vi "CarWashTest.vi"(0 "VI Reference In":refnum<vi>, 2 "Label":string, 5 "Wash Option":string, 7 "Car Position":i32=1, 9 "Elapsed Time":dbl=5.0, 11 "error in":errorcluster) -> (4 "VI Reference Out":refnum<vi>, 15 "error out":errorcluster)   [LabVIEW 2016, in "CarWashTest.lvlib"]
doc: "Wash test"
uses:
  CarWashTest.lvlib
  APIs/Stimulus/VI/OpenVIFrontPanel.vi
  APIs/Stimulus/ControlValue/ValueSignalByPathString.vi
  APIs/Stimulus/ControlValue/ValueSignalLatchBooleanString.vi
  APIs/Assert/AssertControlProperty/AssertControlDisable/AssertDisabledAndGrayedOut.vi
  APIs/Assert/AssertControlValue/True.vi
  APIs/Stimulus/ControlValue/SetValueAuto.vi
  APIs/Assert/AssertControlValue/Equal.vi
  APIs/Assert/AssertControlValue/AlmostEqual.vi
  <vilib>/addons/_JKI Toolkits/Caraya/classes/Assert/Assert Almost Equal_Float.vi
  Drona.lvlib
  <vilib>/addons/_JKI Toolkits/Caraya/classes/Test/Test.lvclass
  APIs/Assert/AssertControlValue/AssertControlValue.lvlib
  <vilib>/addons/_JKI Toolkits/Caraya/classes/Assert/Assert.lvclass
  APIs/Assert/AssertControlProperty/AssertControlDisable/AssertControlDisable.lvlib
  APIs/Stimulus/ControlValue/ControlValue.lvlib
  APIs/Stimulus/VI/VI.lvlib
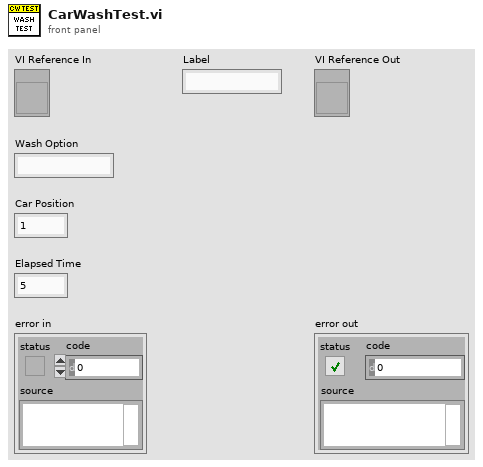
[diagram p1: front panel]
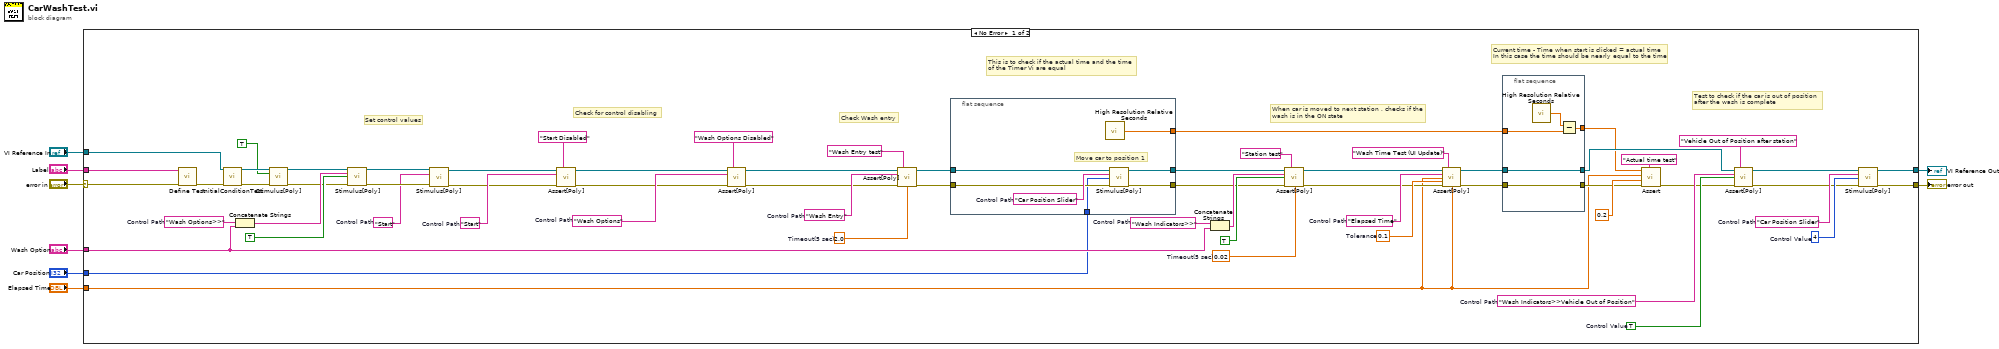
[diagram p0: block diagram]
diagram:
  n1 = case shown="No Error" "error in" {
    selector: "error in" -> [w50 w84]
    tunnel: "Wash Option" -> [w42 _]
    tunnel: "Car Position" -> [w41 _]
    tunnel: "Label" -> [w40 _]
    tunnel: "VI Reference In" -> [w36 _]
    tunnel: "Elapsed Time" -> [w26 _]
    tunnel: [w10 _] -> w2
    tunnel: [w9 w84] -> w1
    frame No Error {
      w19 = "Start"  # Control Path
      w20 = "Wash Options"  # Control Path
      w44 = "Wash Indicators>>"  # Control Path
      w45 = "Start"  # Control Path
      w49 = "Wash Options>>"  # Control Path
      w55 = 4  # Control Value
      w56 = "Car Position Slider"  # Control Path
      w59 = TRUE  # Control Value
      w66 = 0.02  # Timeout(5 sec)
      w63 = 0.1  # Tolerance
      w64 = "Elapsed Time"  # Control Path
      w60 = "Wash Indicators>>Vehicle Out of Position"  # Control Path
      w70 = 2.0  # Timeout(5 sec)
      w71 = "Wash Entry"  # Control Path
      # "Current time - Time when start is clicked = actual time\nIn this case the time should be nearly equal to the time"
      # "This is to check if the actual time and the time \nof the Timer Vi are equal"
      # "Check Wash entry"
      # "Check for control disabling"
      # "Set control values"
      # "Test to check if the car is out of position \nafter the wash is complete"
      # "When car is moved to next station , checks if the\nwash is in the ON state"
      n2 = call <vilib>:"Define Test.vi"("error in (no error)"=w50, "Label (VI Title)"=w40) -> ("error out"=w37:errorcluster)  [unwired: 8 in, 1 out]
      n3 = call "InitialConditionTest.vi"("VI Reference In"=w36, "error in"=w37) -> ("VI Reference Out"=w25:refnum<vi>, "error out"=w23:errorcluster)  [unwired: 12 in]
      n4 = Concatenate Strings(w49, w42) -> (w51:string)
      n5 = call-poly "Stimulus[Poly].vi"("VI Reference In"=w25, "Activate (F)"=TRUE ("Wait Until Done (F)"), "error in"=w23) -> ("VI Reference Out"=w24:refnum<vi>, "error out"=w22:errorcluster)  [unwired: 11 in]
      n6 = call-poly "Stimulus[Poly].vi"("VI Reference In"=w24, "Control Path"=w51, "Value (Signaling)"=TRUE, "error in"=w22) -> ("VI Reference Out"=w47:refnum<vi>, "error out"=w48:errorcluster)  [unwired: 10 in]
      n7 = call-poly "Stimulus[Poly].vi"("VI Reference In"=w47, "Control Path"=w45, "error in"=w48) -> ("VI Reference Out"=w15:refnum<vi>, "error out"=w12:errorcluster)  [unwired: 11 in]
      n8 = call-poly "Assert[Poly].vi"("VI Reference In"=w15, "Test Label"="Start Disabled", "Control Path"=w19, "Error In"=w12) -> ("VI Reference Out"=w17:refnum<vi>, "Error Out"=w18:errorcluster)  [unwired: 9 in, 1 out]
      n9 = call-poly "Assert[Poly].vi"("VI Reference In"=w17, "Test Label"="Wash Options Disabled", "Control Path"=w20, "Error In"=w18) -> ("VI Reference Out"=w14:refnum<vi>, "Error Out"=w13:errorcluster)  [unwired: 9 in, 1 out]
      n10 = call-poly "Assert[Poly].vi"("VI Reference In"=w14, "Test Label"="Wash Entry test" ("Label"), "Control Path"=w71, "Error In"=w13, "Timeout(5 sec)"=w70) -> ("VI Reference Out"=w68:refnum<vi>, "Error Out"=w69:errorcluster)  [unwired: 8 in, 1 out]
      n11 = flat-sequence {
        tunnel: w69 -> [w82]
        tunnel: w68 -> [w81]
        tunnel: [w80] -> w57
        tunnel: w41 -> [w79]
        tunnel: [w78] -> w38
        tunnel: [w77] -> w32
        frame #0 {
          w83 = "Car Position Slider"  # Control Path
          # "Move car to position 1"
          n12 = call <vilib>:"High Resolution Relative Seconds.vi"() -> ("relative seconds"=w77:dbl)
          n13 = call-poly "Stimulus[Poly].vi"("VI Reference In"=w81, "Control Path"=w83, "Value (Signaling)"=w79, "error in"=w82) -> ("VI Reference Out"=w80:refnum<vi>, "error out"=w78:errorcluster)  [unwired: 10 in]
        }
      }
      n14 = Concatenate Strings(w44, w42) -> (w43:string)
      n15 = call-poly "Assert[Poly].vi"("VI Reference In"=w57, "Test Label"="Station test" ("Label"), "Control Path"=w43, "Control Value"=TRUE, "Error In"=w38, "Timeout(5 sec)"=w66) -> ("VI Reference Out"=w62:refnum<vi>, "Error Out"=w39:errorcluster)  [unwired: 7 in, 1 out]
      n16 = call-poly "Assert[Poly].vi"("VI Reference In"=w62, "Test Label"="Wash Time Test (UI Update)" ("Label"), "Control Path"=w64, "Control Value"=w26, "Tolerance"=w63, "Error In"=w39, "Timeout(5 sec)"=w26) -> ("VI Reference Out"=w34:refnum<vi>, "Error Out"=w35:errorcluster)  [unwired: 6 in, 1 out]
      n17 = flat-sequence {
        tunnel: [w76] -> w27
        tunnel: w35 -> [w76]
        tunnel: [w75] -> w33
        tunnel: w34 -> [w75]
        tunnel: w32 -> [w73]
        tunnel: [w72] -> w29
        frame #0 {
          n18 = call <vilib>:"High Resolution Relative Seconds.vi"() -> ("relative seconds"=w74:dbl)
          n19 = Subtract(x=w74, y=w73) -> (x-y=w72:dbl)
        }
      }
      n20 = call-poly <vilib>:"Assert.vi"("Label"="Actual time test", "error in (no error)"=w27, "Tolerance"=0.2, "Y"=w26, "X"=w29) -> ("error out"=w28:errorcluster)  [unwired: 5 in, 1 out]
      n21 = call-poly "Assert[Poly].vi"("VI Reference In"=w33, "Test Label"="Vehicle Out of Position after station" ("Label"), "Control Path"=w60, "Control Value"=w59, "Error In"=w28) -> ("VI Reference Out"=w54:refnum<vi>, "Error Out"=w53:errorcluster)  [unwired: 8 in, 1 out]
      n22 = call-poly "Stimulus[Poly].vi"("VI Reference In"=w54, "Control Path"=w56, "Value (Signaling)"=w55, "error in"=w53) -> ("VI Reference Out"=w10:refnum<vi>, "error out"=w9:errorcluster)  [unwired: 10 in]
    }
    frame Error {
    }
  }
  "error out" <- w1
  "VI Reference Out" <- w2
